vi "FLIR camera_14.1.vi"() -> ()   [LabVIEW 2025]
doc: "The Stream to AVI Files example shows how to save images to an AVI file when using a grab acquisition. This example uses a grab acquisition which works for all camera formats and image sizes. It is recommended to use the Stream to AVI File (Optimized Performance) example if your camera settings work with a ring acquisition."
uses:
  <vilib>/vision/Avi.llb/IMAQ AVI2 Codec Path.ctl
  VIs_needed/Grab Manager Mode.ctl
  <vilib>/vision/Image Controls.llb/IMAQ Image.ctl
  <vilib>/vision/driver/IMAQdx.llb/IMAQdx Buffer Number Mode.ctl
  <vilib>/Utility/High Resolution Relative Seconds.vi
  <vilib>/vision/driver/NI_Vision_Acquisition_Software.lvlib
  <resource>/objmgr/imaqdx.rc
panel:
  out "Boolean":bool
  out "Image":T1(plugin-control)
  out "stripped path":path
  in  "Skip Count":u32
  out "Images Saved Per Second":dbl
  out "Images Acquired Per Second":dbl
  in  "Images per AVI":i32=100
  out "Write Speed":dbl(graph) caption="Image File Write Speed"
  in  "Start":bool
  in  "Codec":u16(ring) items=["FF Video Codec 1 (FFV1) (NI Vision)", "Motion JPEG (NI Vision)", "VP8 (NI Vision)", "VP9 (NI Vision)", "Y800 Uncompressed Grey Scale (NI Vision)", "YUV 4:2:0 Planar (NI Vision)"]
  out "Destination Folder":path
  out "Images Behind":i32
  in  "Number of Images":u32=30
  in  "Camera Name":refnum<k21> caption="IMAQdx Session"
  in  "Stop":bool
  # "Overview: Demonstrates how to stream images to an AVI file when using a grab acquisition.\nRequirements: Vision Acquisition Software\nInstructions:\n1. Select the Camera Name\n2. Run the VI\n3. Select the Codec and click Start.\n4. Increase the Skip Count if Images Behind is greater than 0."
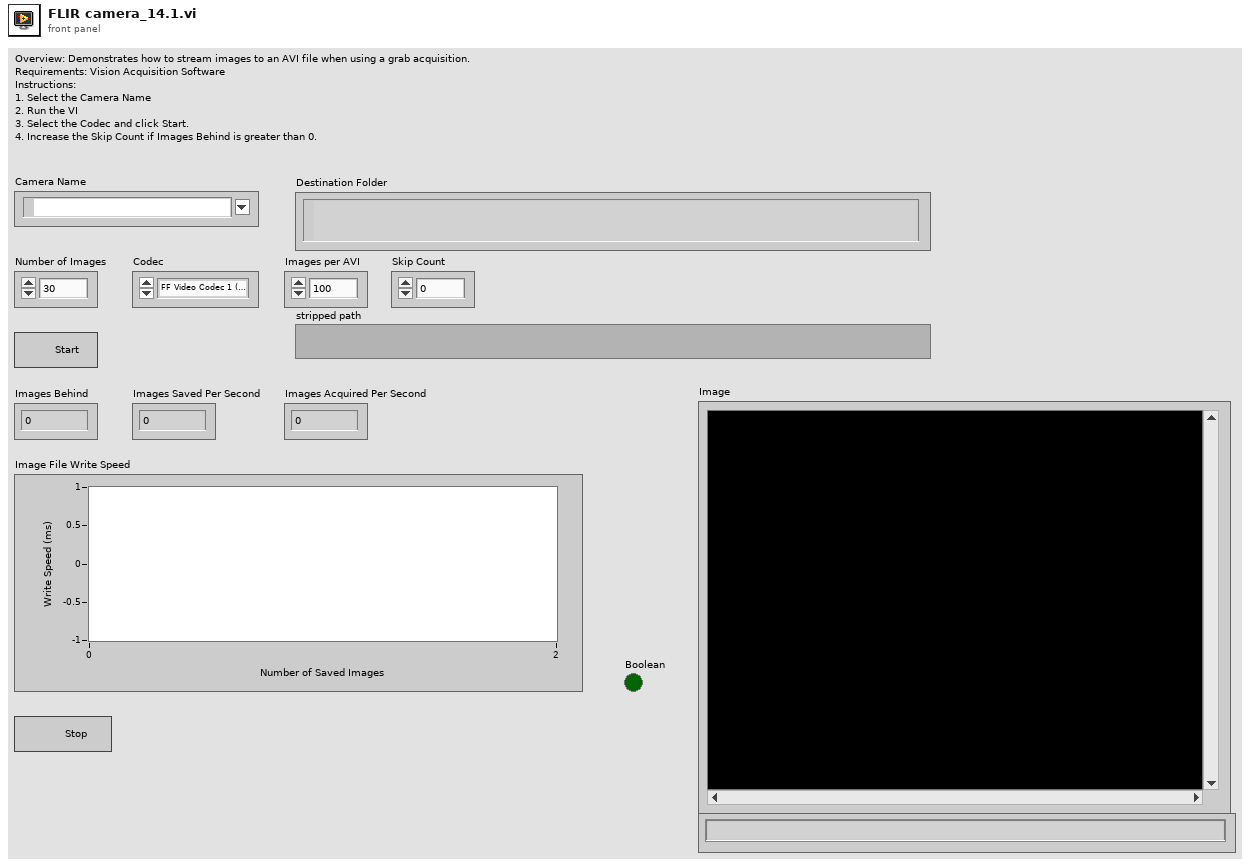
[diagram p1: front panel]
types:
  T1 = typedef "IMAQ Image.ctl" = refnum<image>
  T2 = typedef "IMAQ AVI2 Codec Path.ctl" = u32
  T3 = typedef "IMAQdx.ctl" = refnum<k21>
  T4 = typedef "Grab Manager Mode.ctl" = enum16{"Create Processing Images", "Lock", "Add Acquired Image", "Get Acquired Image", "Unlock", "Dispose Processing Images"}
  T5 = cluster{"Number of Processing Images":u32, "Image Border Size":u32}
  T6 = typedef "NI_Vision_Acquisition_Software.lvlib/IMAQdx Buffer Number Mode.ctl" = enum32{"Next", "Last", "Buffer Number", "Every", "Last New"}
  T7 = typedef "IMAQ AVI2 Refnum.ctl" = refnum<k20>
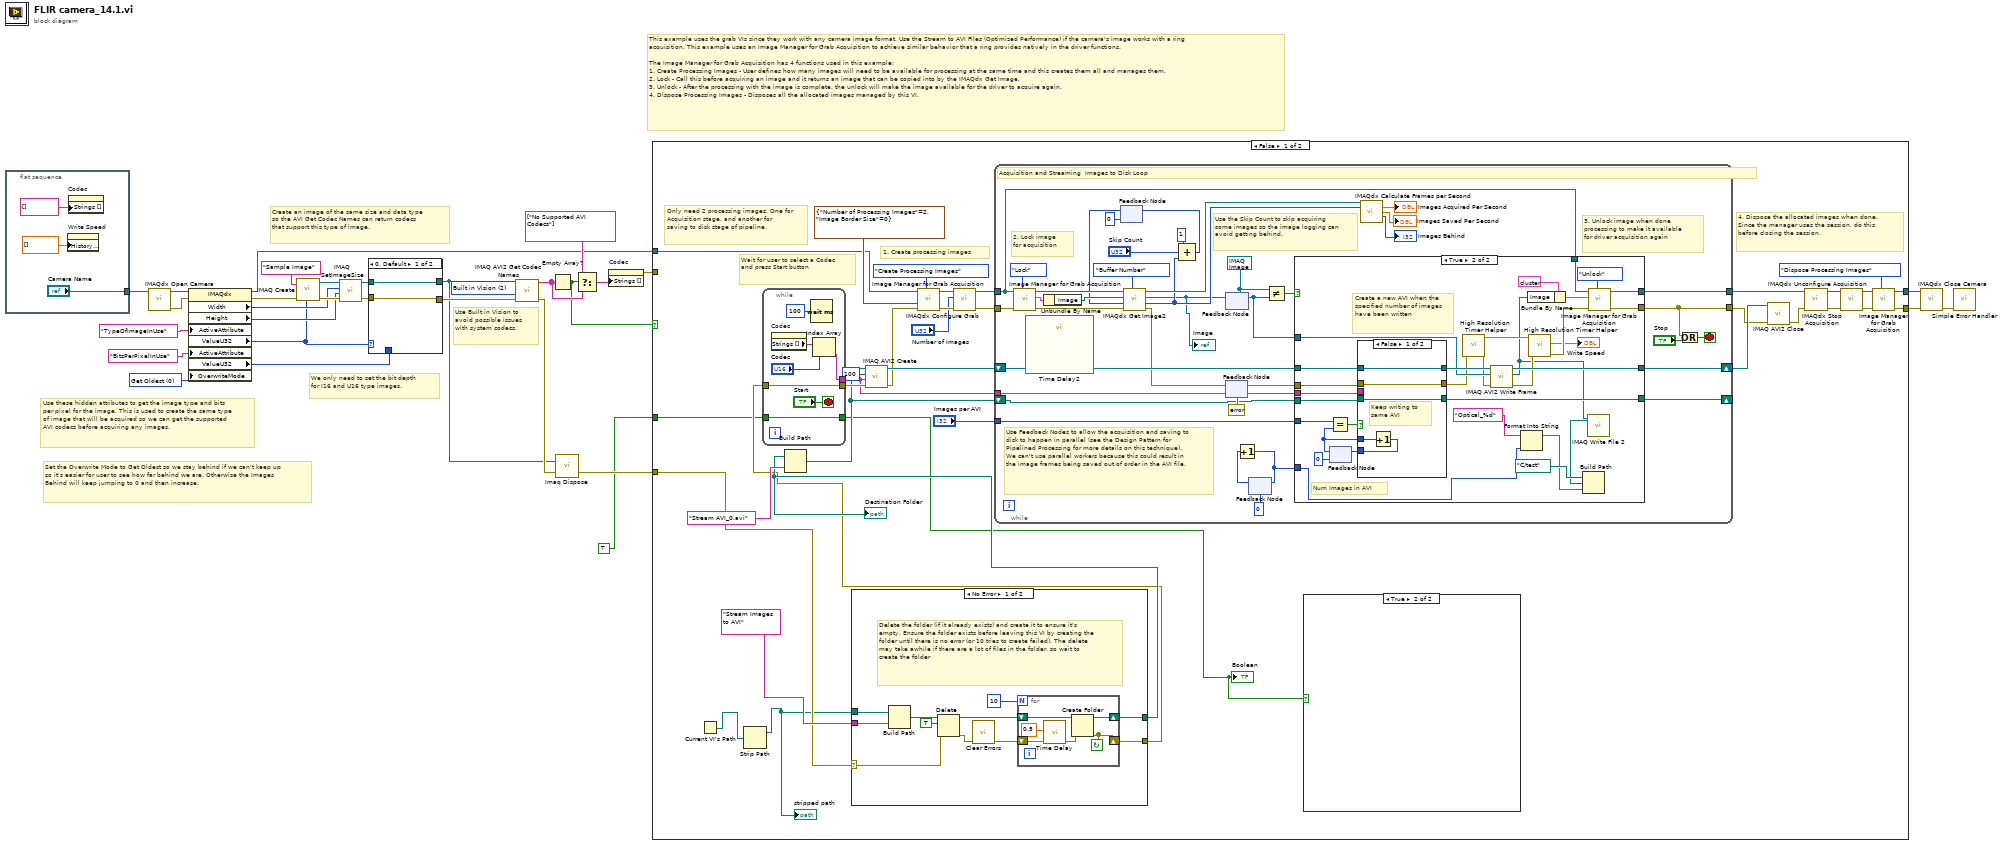
[diagram p0: block diagram]
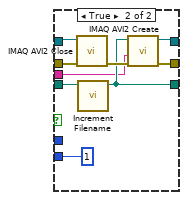
[diagram p5: hidden frame]
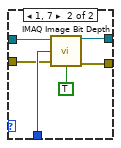
[diagram p7: hidden frame]
diagram:
  w2 = T2 2 items=["Default", "System", "Built in Vision"] ("Codec Source")
  w4 = u32 0 items=["Get Oldest"=0, "Fail"=2, "Get Newest"=3] ("OverwriteMode")
  # "Use Built in Vision to avoid possible issues with system codecs."
  # "This example uses the grab VIs since they work with any camera image format. Use the Stream to AVI Files (Optimized Performance) if the camera's image works with a ring acquisition. This example uses an Image Manager for Grab Acquisition to achieve similar behavior that a ring provides natively in the driver functions.\n\nThe Image Manager for Grab Acquisition has 4 functions used in this example:\n1. Create Processing Images - User defines how many images will need to be available for processing at the same time and this creates them all and manages them.\n2. Lock - Call this before acquiring an image and it returns an image that can be copied into by the IMAQdx Get Image.\n3. Unlock - After the processing with the image is complete, the unlock will make the image available for the driver to acquire again.\n4. Dispose Processing Images - Disposes all the allocated images managed by this VI."
  # "Set the Overwrite Mode to Get Oldest so we stay behind if we can't keep up so it's easier for user to see how far behind we are. Otherwise the Images Behind will keep jumping to 0 and then increase."
  # "Create an image of the same size and data type so the AVI Get Codec Names can return codecs that support this type of image."
  # "Use these hidden attributes to get the image type and bits per pixel for the image. This is used to create the same type of image that will be acquired so we can get the supported AVI codecs before acquiring any images."
  # "We only need to set the bit depth for I16 and U16 type images."
  n1 = flat-sequence {
    tunnel: ["Camera Name"] -> w31
    frame #0 {
      n2 = property on="Write Speed" class="WFChart (strict)"("History Data"=dbl[] []) -> ()  [unwired: 2 in, 2 out]
      n3 = property on="Codec" class="Ring (strict)"("Strings []"=string[] []) -> ()  [unwired: 2 in, 2 out]
    }
  }
  n4 = call <vilib>:"IMAQdx Open Camera.vi"("Session In"=w31) -> ("error out"=w27:errorcluster, "Session Out"=w28:T3)  [unwired: 2 in, 7 out]
  n5 = property class="IMAQdx"(reference=w28, error in=w27, "ActiveAttribute"="TypeOfImageInUse", "ActiveAttribute"="BitsPerPixelInUse", "OverwriteMode"=w4) -> (reference out=w13:T3, error out=w25:errorcluster, "Width"=w21:u32, "Height"=w20:u32, "ValueU32"=w8:u32, "ValueU32"=w11:u32)
  n6 = call "IMAQ Create"("Image Name"="Sample Image", "Image Type"=w8, "error in (no error)"=w25) -> ("New Image"=w22:T1, "error out"=w23:errorcluster)  [unwired: 1 in, 1 out]
  n7 = call "IMAQ SetImageSize"("error in (no error)"=w23, "Y Resolution"=w20, "X Resolution"=w21, "Image"=w22) -> ("error out"=w10:errorcluster, "Image Out"=w9:T1)  [unwired: 1 in]
  n8 = case shown="0, Default" w8 {
    tunnel: [w35 w42] -> w14
    tunnel: w11 -> [_ w41]
    tunnel: w10 -> [w35 w40]
    tunnel: w9 -> [w36 w38]
    tunnel: [w36 w37] -> w5
    frame 0, Default {
    }
    frame 1, 7 {
      n9 = call "IMAQ Image Bit Depth"("Image"=w38, "Bit Depth (0)"=w41, "error in (no error)"=w40, "Get/Set Bit Depth? (Set)"=TRUE) -> ("Image Out"=w37:T1, "error out"=w42:errorcluster)  [unwired: 9 in, 1 out]
    }
  }
  n10 = call "IMAQ AVI2 Get Codec Names"("error in (no error)"=w14, "Codec Source"=w2, "Image"=w5) -> ("error out"=w7:errorcluster, "Codec Names"=w19:string[])  [unwired: 7 in]
  n11 = Empty Array?(array=w19) -> (empty?=w15:bool)
  n12 = call "Imaq Dispose"("Image"=w5, "error in (no error)"=w7) -> ("error out"=w6:errorcluster)  [unwired: 4 in]
  n13 = Select(t=string[] ["No Supported AVI Codecs"], s=w15, f=w19) -> (s? t:f=w17:string[])
  n14 = property on="Codec" class="Ring (strict)"("Strings []"=w17) -> (error out=w16:errorcluster)  [unwired: 2 in, 1 out]
  n15 = case shown="False" w15 {
    tunnel: [w53 w190] -> w30
    tunnel: [w54 w191] -> w29
    tunnel: w13 -> [w59 w191]
    tunnel: w6 -> [w50 w190]
    tunnel: w16 -> [_ _]
    tunnel: TRUE -> [w45 _]
    frame False {
      # "4. Dispose the allocated images when done. Since the manager uses the session, do this before closing the session."
      # "1. Create processing images"
      # "Only need 2 processing images. One for Acquisition stage, and another for saving to disk stage of pipeline."
      # "Wait for user to select a Codec and press Start button"
      n16 = Current VI's Path() -> (path=w47:path)
      n17 = Strip Path(path=w47) -> (stripped path=w46:path)  [unwired: 1 out]
      "stripped path" <- w46
      n18 = case shown="No Error" w50 {
        selector: w50 -> [w79 w95]
        tunnel: w46 -> [w88 _]
        tunnel: [w81 _] -> w49
        tunnel: "Stream Images to AVI" ("Folder Name") -> [w80 _]
        tunnel: [w78 w95] -> w48
        frame No Error {
          # "Delete the folder (if it already exists) and create it to ensure it's empty. Ensure the folder exists before leaving this VI by creating the folder until there is no error (or 10 tries to create failed). The delete may take awhile if there are a lot of files in the folder, so wait to create the folder"
          n19 = Build Path(base path=w88, name or relative path=w80) -> (appended path=w86:path)
          n20 = Delete(path (use dialog)=w86, entire hierarchy (F)=TRUE, error in=w79) -> (deleted path=w85:path, error out=w84:errorcluster)  [unwired: 2 in, 1 out]
          n21 = call <vilib>:"Clear Errors.vi"("error in (no error)"=w84) -> ("error out"=w83:errorcluster)  [unwired: 5 in, 1 out]
          n22 = for {
            N: 10 -> [_]
            shift-right: [w93] -> w81
            shift-left: w85 -> [w94]
            shift-right: [w92] -> w78
            shift-left: w83 -> [w91]
            stop <- w92 continue-if-true
            n23 = call "Time Delay"("error in (no error)"=w91, "Delay Time (s)"=0.5) -> ("error out"=w90:errorcluster)  [unwired: 9 in]
            n24 = Create Folder(path (use dialog)=w94, error in=w90) -> (created path=w93:path, error out=w92:errorcluster)  [unwired: 2 out]
          }
        }
        frame Error {
        }
      }
      "Destination Folder" <- w49
      n25 = while {
        tunnel: w48 -> [w188]
        tunnel: [w188] -> w74
        tunnel: [w185] -> w66
        tunnel: [w183] -> w44
        tunnel: w45 -> [w183]
        stop <- "Start" stop-if-true
        n26 = property on="Codec" class="Ring (strict)"() -> ("Strings []"=w186:string[])  [unwired: 2 in, 2 out]
        n27 = Wait (ms)(milliseconds to wait=u32 100) -> ()  [unwired: 1 out]
        n28 = Index Array(array=w186, index="Codec") -> (element=w185:string)
      }
      "Boolean" <- w44
      n29 = Build Path(base path=w49, name or relative path="Stream AVI_0.avi") -> (appended path=w67:path)
      n30 = call "IMAQ AVI2 Create"("error in (no error)"=w74, "Codec"=w66, "Frames Per Second"=u32 100, "AVI Path"=w67) -> ("error out"=w58:errorcluster, "AVI Refnum"=w69:T7)  [unwired: 6 in]
      n31 = call "Image Manager for Grab Acquisition.vi"("Mode"=Grab_Manager_Mode."Create Processing Images", "error in (no error)"=w58, "Init Settings"=T5 {"Number of Processing Images"=2, "Image Border Size"=0}, "Session In"=w59) -> ("error out"=w61:errorcluster, "Session Out"=w60:T3)  [unwired: 4 in, 2 out]
      n32 = call <vilib>:"IMAQdx Configure Grab.vi"("error in"=w61, "Number of Buffers"="Number of Images", "Session In"=w60) -> ("error out"=w64:errorcluster, "Session Out"=w65:T3)  [unwired: 7 in]
      n33 = while {
        tunnel: w64 -> [w118]
        tunnel: w65 -> [w119]
        tunnel: [w131] -> w75
        tunnel: [w125] -> w72
        shift-right: [w132] -> w73
        shift-left: w69 -> [w124]
        tunnel: "Images per AVI" -> [w121]
        shift-right: [w122] -> _
        shift-left: w67 -> [w101]
        tunnel: w66 -> [w123]
        stop <- w127 stop-if-true
        w129 = T1 refnum ("Image Out")
        # "3. Unlock image when done processing to make it available for driver acquisition again"
        # "2. Lock image for acquisition"
        # "Use the Skip Count to skip acquiring some images so the image logging can avoid getting behind."
        # "Use Feedback Nodes to allow the acquisition and saving to disk to happen in parallel (see the Design Pattern for Pipelined Processing for more details on this technique). We can't use parallel workers because this could result in the image frames being saved out of order in the AVI file."
        # "Acquisition and Streaming  Images to Disk Loop"
        n34 = call "Image Manager for Grab Acquisition.vi"("Mode"=Grab_Manager_Mode."Lock", "error in (no error)"=w118, "Session In"=w119) -> ("error out"=w115:errorcluster, "Image Settings Out"=w113:cluster{"Image":T1, "Buffer Number":u32}, "Session Out"=w116:T3)  [unwired: 5 in, 1 out]
        n35 = call "Time Delay2"() -> ()  [unwired: 11 in, 1 out]
        n36 = Unbundle By Name(w113) -> ("Image"=w112:T1)
        n37 = feedback #1(u32 0) -> (w109:u32)
        n38 = call <vilib>:"IMAQdx Get Image2.vi"("Buffer Number Mode (Next)"=IMAQdx_Buffer_Number_Mode."Buffer Number", "error in"=w115, "Buffer Number In"=w109, "Image In"=w112, "Session In"=w116) -> ("error out"=w111:errorcluster, "Buffer Number Out"=w105:u32, "Image Out"=w100:T1, "Session Out"=w110:T3)  [unwired: 3 in]
        "Image" <- w100
        n39 = Compound Arithmetic op=ADD(u32 1, "Skip Count", w105) -> (w104:u32)
        n40 = feedback-in #1(w104) -> ()
        n41 = feedback-in #2(w111) -> ()
        n42 = feedback #2(errorcluster {"status"=FALSE, "code"=0, "source"=""} ("error out")) -> (w130:errorcluster)
        n43 = feedback-in #3(w100) -> ()
        n44 = feedback #3(w129) -> (w99:T1)
        n45 = feedback #4(0) -> (w97:i32)
        n46 = Increment(x=w97) -> (x+1=w96:i32)
        n47 = feedback-in #4(w96) -> ()
        n48 = Not Equal?(x=w129, y=w99) -> (x != y?=w128:bool)
        n49 = case shown="True" w128 {
          tunnel: w124 -> [w135 w163]
          tunnel: w99 -> [_ w158]
          tunnel: w130 -> [w136 w162]
          tunnel: [w135 w168] -> w132
          tunnel: [w137 w152] -> w131
          tunnel: w119 -> [w137 w149]
          tunnel: [w136 w151] -> w125
          tunnel: w123 -> [_ w161]
          tunnel: w101 -> [w134 w144]
          tunnel: [w134 w159] -> w122
          tunnel: w121 -> [_ w157]
          tunnel: w96 -> [_ w141]
          frame False {
            # "First iteration doesn't have valid image for this pipelined stage."
          }
          frame True {
            # "Create a new AVI when the specified number of images have been written"
            # "Num Images in AVI"
            n50 = feedback #5(0) -> (w167:i32)
            n51 = Equal?(x=w157, y=w167) -> (x = y?=w164:bool)
            n52 = case shown="False" w164 {
              tunnel: [w172 1] -> w166
              tunnel: w167 -> [w173 _]
              tunnel: w163 -> [w171 w180]
              tunnel: [w171 w177] -> w160
              tunnel: w144 -> [w169 w181]
              tunnel: w162 -> [w170 w179]
              tunnel: [w170 w176] -> w156
              tunnel: [w169 w175] -> w159
              tunnel: w161 -> [_ w174]
              frame False {
                # "Keep writing to same AVI"
                n53 = Increment(x=w173) -> (x+1=w172:i32)
              }
              frame True {
                n54 = call "IMAQ AVI2 Close"("error in (no error)"=w179, "AVI Refnum"=w180) -> ("error out"=w178:errorcluster)  [unwired: 9 in]
                n55 = call "Increment Filename.vi"("Path In"=w181) -> ("Incremented Path Out"=w175:path)  [unwired: 10 in]
                n56 = call "IMAQ AVI2 Create"("error in (no error)"=w178, "Codec"=w174, "AVI Path"=w175) -> ("error out"=w176:errorcluster, "AVI Refnum"=w177:T7)  [unwired: 7 in]
              }
            }
            n57 = feedback-in #5(w166) -> ()
            n58 = call "High Resolution Timer Helper.vi"("error in (no error)"=w156) -> ("error out"=w155:errorcluster, "Current Time"=w153:dbl)  [unwired: 8 in, 1 out]
            n59 = call "IMAQ AVI2 Write Frame"("error in (no error)"=w155, "Image"=w158, "AVI Refnum"=w160) -> ("error out"=w154:errorcluster, "Image Out (duplicate)"=w143:T1, "AVI Refnum (duplicate)"=w168:T7)  [unwired: 6 in]
            n60 = Format Into String(initial string="Optical_%d", w141) -> (resulting string=w139:string)  [unwired: 2 in, 1 out]
            n61 = Bundle By Name(cluster=cluster{"Image":T1, "Buffer Number":u32} {"Image"=refnum, "Buffer Number"=0} ("Image Settings In"), "Image"=w143) -> (w146:cluster{"Image":T1, "Buffer Number":u32})
            n62 = call "High Resolution Timer Helper.vi"("error in (no error)"=w154, "Previous Time"=w153) -> ("error out"=w150:errorcluster, "Time Difference (ms)"=→"Write Speed":dbl)  [unwired: 7 in, 1 out]
            n63 = Build Path(base path=path "C:/test", name or relative path=w139) -> (appended path=w138:path)
            n64 = call-poly "IMAQ Write File 2"("File Path"=w138, "Image"=w143) -> ()  [unwired: 8 in, 2 out]
            n65 = call "Image Manager for Grab Acquisition.vi"("Mode"=Grab_Manager_Mode."Unlock", "error in (no error)"=w150, "Image Settings In"=w146, "Session In"=w149) -> ("error out"=w151:errorcluster, "Session Out"=w152:T3)  [unwired: 4 in, 2 out]
          }
        }
        n66 = call <vilib>:"IMAQdx Calculate Frames per Second.vi"("Session In"=w110, "Buffer Number"=w105) -> ("Acquired Frames per Second"=→"Images Acquired Per Second":dbl, "Processed Frames per Second"=→"Images Saved Per Second":dbl, "Images Behind"=→"Images Behind":i32)  [unwired: 7 in, 4 out]
        n67 = Or(x=w125, y="Stop") -> (x .or. y?=w127:bool)
      }
      n68 = case shown="True" w44 {
        frame False {
        }
        frame True {
        }
      }
      n69 = call "IMAQ AVI2 Close"("error in (no error)"=w72, "AVI Refnum"=w73) -> ("error out"=w71:errorcluster)  [unwired: 9 in]
      n70 = call <vilib>:"IMAQdx Stop Acquisition.vi"("error in"=w71, "Session In"=w75) -> ("error out"=w76:errorcluster, "Session Out"=w77:T3)  [unwired: 8 out]
      n71 = call <vilib>:"IMAQdx Unconfigure Acquisition.vi"("error in"=w76, "Session In"=w77) -> ("error out"=w57:errorcluster, "Session Out"=w56:T3)  [unwired: 8 out]
      n72 = call "Image Manager for Grab Acquisition.vi"("Mode"=Grab_Manager_Mode."Dispose Processing Images", "error in (no error)"=w57, "Session In"=w56) -> ("error out"=w53:errorcluster, "Session Out"=w54:T3)  [unwired: 5 in, 2 out]
    }
    frame True {
      # "No valid AVI Codecs for the image size and image type."
    }
  }
  n73 = call <vilib>:"IMAQdx Close Camera.vi"("error in"=w30, "Session In"=w29) -> ("error out"=w3:errorcluster)  [unwired: 9 out]
  n74 = call <vilib>:"Simple Error Handler.vi"("error in (no error)"=w3) -> ()  [unwired: 4 in, 5 out]
